vi "run_tests.vi"(11 "Command Line":string[](array[string])) -> (2 "stdout | stderr":string, 3 "Return Code":i32)   [LabVIEW 2021]
uses:
  <vilib>/Utility/error.llb/DialogType.ctl
  20ab466a-1420-47d7-bd04-4ec556d045c0.vi
  <vilib>/Utility/error.llb/Error Cluster From Error Code.vi
  <vilib>/Comparison/Equal/Equal Functor/Equal Functor.lvclass
  <vilib>/ErrorRing/Error Ring.xnode
panel:
  out "Any Failures?":bool
  out "Live results":string
  out "Current Test\nSucceeded":bool
  out "Current":i32
  out "Total":i32
  out "Current Test":path
  out "Full Report":string
  out "All Tests Passed":bool
  out "error out":errorcluster
  # "Required by LabVIEWCLI\n(via connector pane)"
  # "Of"
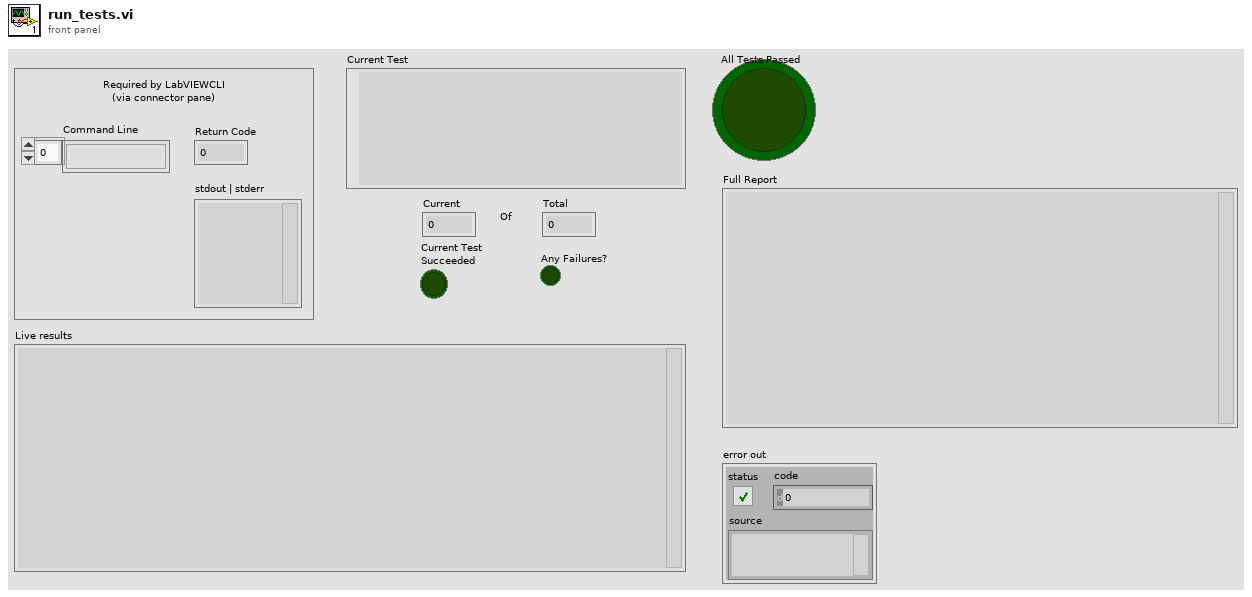
[diagram p1: front panel]
types:
  T1 = typedef "DialogType.ctl" = u16
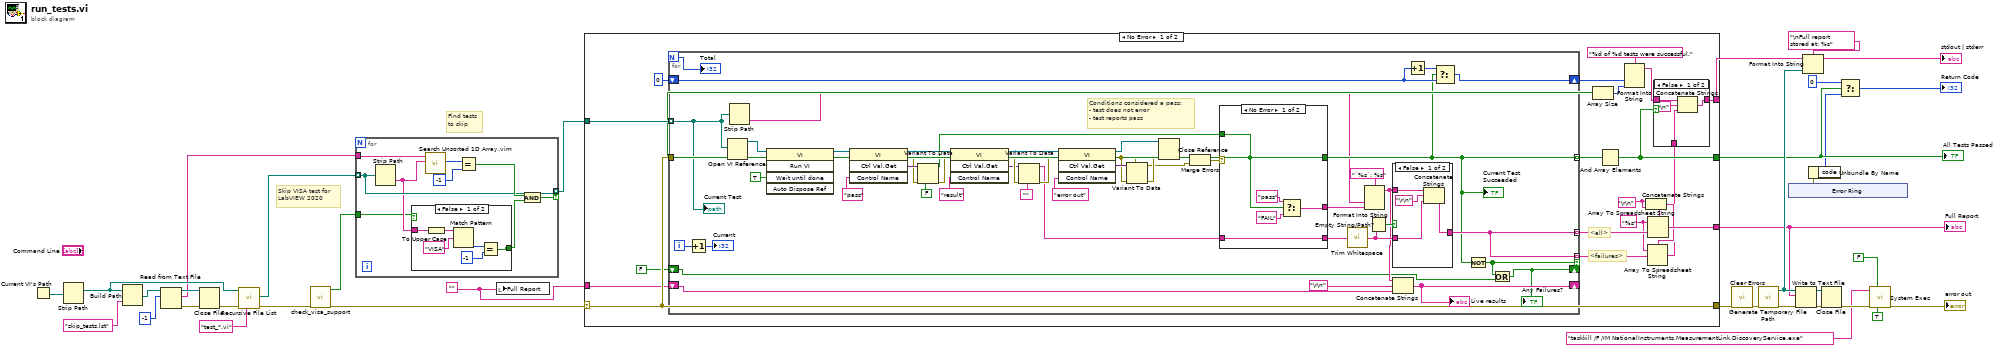
[diagram p0: block diagram]
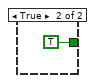
[diagram p2: hidden frame]
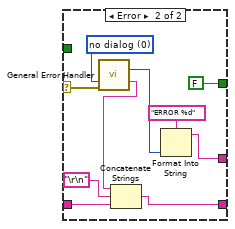
[diagram p5: hidden frame]
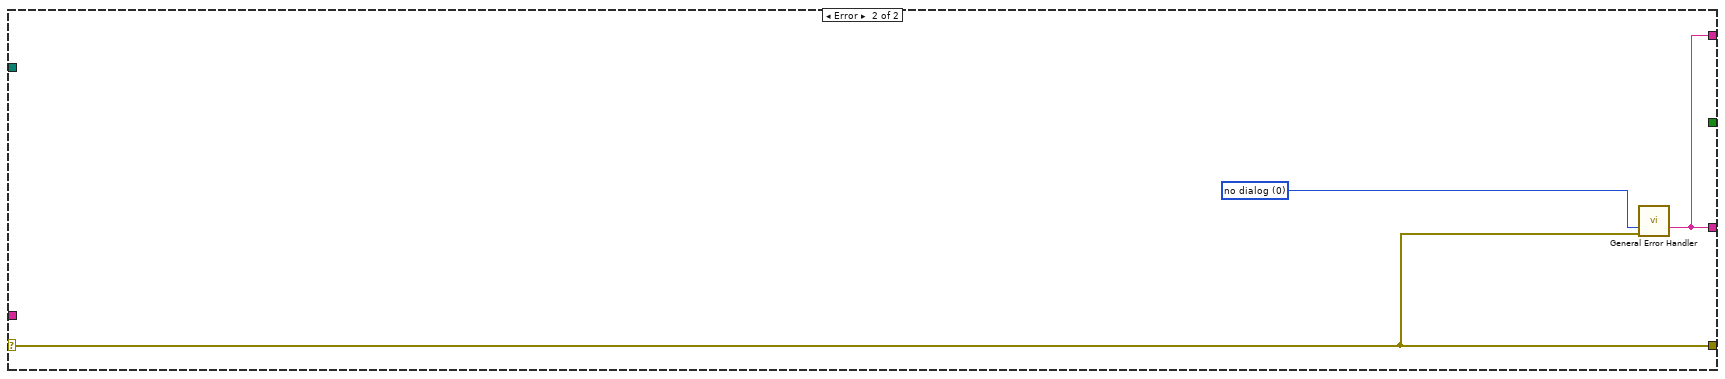
[diagram p6: hidden frame]
diagram:
  w1 = ""
  # "Skip VISA test for LabVIEW 2020"
  # "Find tests\nto skip"
  n1 = Current VI's Path() -> (path=w36:path)
  n2 = Strip Path(path=w36) -> (stripped path=w16:path)  [unwired: 1 out]
  n3 = Build Path(base path=w16, name or relative path="skip_tests.lst") -> (appended path=w14:path)
  n4 = Read from Text File(file (use dialog)=w14, count=-1) -> (refnum out=w17:refnum<file>, text=w11:string[], error out=w19:errorcluster)  [unwired: 2 in, 1 out]
  n5 = Close File(refnum=w17, error in=w19) -> (error out=w18:errorcluster)  [unwired: 1 out]
  n6 = call <vilib>:"Recursive File List.vi"("pattern"="test_*.vi", "error in (no error)"=w18, "Folder Path"=w16) -> ("error out"=w8:errorcluster, "All Files in Dir"=w12:path[])  [unwired: 4 in, 3 out]
  n7 = call "check_visa_support.vi"("error in"=w8) -> ("error out"=w2:errorcluster, "visa supported"=w9:bool)  [unwired: 9 in]
  n8 = for {
    tunnel: w12 -> [w40] mode=indexing
    tunnel: w11 -> [w45]
    tunnel: [w40] -> w10 mode=indexing if=w42
    tunnel: w9 -> [w37]
    n9 = Strip Path(path=w40) -> (name=w38:string)  [unwired: 1 out]
    n10 = case shown="False" w37 {
      tunnel: [w46 TRUE] -> w39
      tunnel: w38 -> [w47 _]
      frame False {
        n11 = To Upper Case(1:w47) -> (0:w51:string)
        n12 = Match Pattern(string=w51, regular expression="VISA") -> (offset past match=w50:i32)  [unwired: 1 in, 3 out]
        n13 = Equal?(x=w50, y=-1) -> (x = y?=w46:bool)
      }
      frame True {
      }
    }
    n14 = call "Search Unsorted 1D Array.vim"("element"=w38, "unsorted 1D array"=w45) -> ("index of element"=w44:i32)  [unwired: 9 in]
    n15 = Equal?(x=w44, y=-1) -> (x = y?=w43:bool)
    n16 = And(x=w43, y=w39) -> (x .and. y?=w42:bool)
  }
  n17 = local write "Full Report"(w1) -> ()
  n18 = case shown="No Error" w2 {
    selector: w2 -> [w70 w149]
    tunnel: w10 -> [w71 _]
    tunnel: [w70 w149] -> w34
    tunnel: [w63 _] -> w25
    tunnel: [w60 w147] -> w26
    tunnel: [w61 w147] -> w31
    tunnel: w1 -> [w54 _]
    frame No Error {
      w56 = "%s" ("format string")
      w69 = "\r\n"
      # "<failures>"
      # "<all>"
      n19 = for {
        N -> [w88]
        tunnel: w71 -> [w89] mode=indexing
        tunnel: w70 -> [w126]
        tunnel: [w91] -> w65 mode=indexing
        tunnel: [w94] -> w59 mode=indexing
        tunnel: [w94] -> w58 mode=indexing if=w79
        shift-right: [w90] -> w66
        shift-left: 0 -> [w92]
        shift-right: [w82] -> _
        shift-left: w54 -> [w81]
        shift-right: [w77] -> _
        shift-left: FALSE -> [w78]
        i -> [w87]
        # "Conditions considered a pass:\n- test does not error\n- test reports pass"
        n20 = Increment(x=w87) -> (x+1=→"Current":i32)
        n21 = Open VI Reference(vi path=w89, error in (no error)=w126) -> (vi reference=w125:refnum<vi>, error out=w124:errorcluster)  [unwired: 4 in]
        n22 = Strip Path(path=w89) -> (name=w85:string)  [unwired: 1 out]
        n23 = invoke class="VI" method="Run VI"(reference=w125, error in=w124, "Wait until done"=TRUE ("Wait Until Done")) -> (reference out=w122:refnum<vi>, error out=w121:errorcluster)  [unwired: 2 in, 3 out]
        n24 = invoke class="VI" method="Ctrl Val.Get"(reference=w122, error in=w121, "Control Name"="pass") -> (reference out=w111:refnum<vi>, error out=w118:errorcluster, "Get Control Value Variant"=w119:variant)  [unwired: 1 in, 1 out]
        n25 = Variant To Data(error in=w118, type=FALSE, Variant=w119) -> (data=w100:bool, error out=w115:errorcluster)
        n26 = invoke class="VI" method="Ctrl Val.Get"(reference=w111, error in=w115, "Control Name"="result") -> (reference out=w106:refnum<vi>, error out=w116:errorcluster, "Get Control Value Variant"=w113:variant)  [unwired: 1 in, 1 out]
        n27 = Variant To Data(error in=w116, type="", Variant=w113) -> (data=w98:string, error out=w109:errorcluster)
        n28 = invoke class="VI" method="Ctrl Val.Get"(reference=w106, error in=w109, "Control Name"="error out") -> (reference out=w105:refnum<vi>, error out=w107:errorcluster, "Get Control Value Variant"=w110:variant)  [unwired: 1 in, 1 out]
        n29 = Variant To Data(error in=w107, type=w107, Variant=w110) -> (data=w102:errorcluster, error out=w108:errorcluster)
        n30 = Close Reference(reference=w105, error in (no error)=w108) -> (error out=w103:errorcluster)
        n31 = Merge Errors(w103, w102) -> (w101:errorcluster)
        n32 = case shown="No Error" w101 {
          selector: w101 -> [_ w144]
          tunnel: w100 -> [w134 _]
          tunnel: [w133 w141] -> w84
          tunnel: [w134 FALSE] -> w91
          tunnel: w98 -> [w132 w140]
          tunnel: [w132 w139] -> w97
          frame No Error {
            n33 = Select(t="pass" ("Control Name"), s=w134, f="FAIL" ("Control Name")) -> (s? t:f=w133:string)
          }
          frame Error {
            w145 = T1 0 items=["no dialog", "OK message", "continue or stop message", "OK message + warnings", "continue/stop + warnings"] ("type of dialog (OK msg:1)")
            n34 = call <vilib>:"General Error Handler.vi"("type of dialog (OK msg:1)"=w145, "error in (no error)"=w144) -> ("code out"=w143:i32, "message"=w138:string)  [unwired: 9 in, 3 out]
            n35 = Concatenate Strings(w138, "\r\n", w140) -> (w139:string)
            n36 = Format Into String(format string="ERROR %d", w143) -> (resulting string=w141:string)  [unwired: 2 in, 1 out]
          }
        }
        "Current Test\nSucceeded" <- w91
        n37 = call <vilib>:"Trim Whitespace.vi"("string"=w97) -> ("trimmed string"=w96:string)  [unwired: 1 in]
        n38 = Format Into String(format string="`%s`: %s" ("Control Name"), w85, w84) -> (resulting string=w80:string)  [unwired: 2 in, 1 out]
        n39 = Empty String/Path?(string/path=w96) -> (empty?=w95:bool)
        n40 = case shown="False" w95 {
          tunnel: w96 -> [w129 _]
          tunnel: w80 -> [w130 w131]
          tunnel: [w128 w131] -> w94
          frame False {
            n41 = Concatenate Strings(w130, "\r\n", w129) -> (w128:string)
          }
          frame True {
          }
        }
        n42 = Concatenate Strings(w80, "\r\n", w81) -> (w82:string)
        "Live results" <- w82
        n43 = Increment(x=w92) -> (x+1=w93:i32)
        n44 = Select(t=w93, s=w91, f=w92) -> (s? t:f=w90:i32)
        n45 = Not(x=w91) -> (.not. x?=w79:bool)
        n46 = Or(x=w79, y=w78) -> (x .or. y?=w77:bool)
        "Any Failures?" <- w77
        "Current Test" <- w89
        "Total" <- w88
      }
      n47 = Array Size(array=w65) -> (size(s)=w64:i32)
      n48 = And Array Elements(Boolean array=w65) -> (logical AND=w63:bool)
      n49 = Format Into String(format string="%d of %d tests were successful." ("Control Name"), w66, w64) -> (resulting string=w62:string)  [unwired: 2 in, 1 out]
      n50 = Concatenate Strings(w69, w69) -> (w57:string)
      n51 = Array To Spreadsheet String(delimiter (Tab)=w57, array=w58, 3:w56) -> (spreadsheet string=w55:string)
      n52 = Array To Spreadsheet String(delimiter (Tab)=w57, array=w59, 3:w56) -> (spreadsheet string=w60:string)
      n53 = case shown="False" w63 {
        tunnel: w62 -> [w75 w76]
        tunnel: [w72 w76] -> w61
        tunnel: w55 -> [w73 _]
        frame False {
          n54 = Concatenate Strings(w75, "\r\n", w73) -> (w72:string)
        }
        frame True {
        }
      }
    }
    frame Error {
      w148 = T1 0 items=["no dialog", "OK message", "continue or stop message", "OK message + warnings", "continue/stop + warnings"] ("type of dialog (OK msg:1)")
      n55 = call <vilib>:"General Error Handler.vi"("type of dialog (OK msg:1)"=w148, "error in (no error)"=w149) -> ("message"=w147:string)  [unwired: 9 in, 4 out]
    }
  }
  "All Tests Passed" <- w25
  "Full Report" <- w26
  n56 = call <vilib>:"Clear Errors.vi"("error in (no error)"=w34) -> ("error out"=w33:errorcluster)  [unwired: 5 in, 1 out]
  n57 = call <vilib>:"Generate Temporary File Path.vi"("error in (no error)"=w33) -> ("error out"=w28:errorcluster, "Unique Temporary File Path"=w29:path)  [unwired: 9 in]
  n58 = xnode "Error Ring"() -> ("error out"=w21:errorcluster)
  n59 = Write to Text File(file (use dialog)=w29, text=w26, error in=w28) -> (refnum out=w30:refnum<file>, error out=w27:errorcluster)  [unwired: 1 in, 1 out]
  n60 = Format Into String(format string="\nFull report stored at: %s" ("Control Name"), initial string=w31, w29) -> (resulting string=→"stdout | stderr":string)  [unwired: 1 in, 1 out]
  n61 = Unbundle By Name(w21) -> ("code"=w20:i32)
  n62 = Close File(refnum=w30, error in=w27) -> (error out=w7:errorcluster)  [unwired: 1 out]
  n63 = Select(t=0, s=w25, f=w20) -> (s? t:f=→"Return Code":i32)
  n64 = call <vilib>:"System Exec.vi"("run minimized? (F)"=TRUE, "wait until completion? (T)"=FALSE, "error in (no error)"=w7, "command line"="taskkill /F /IM NationalInstruments.MeasurementLink.DiscoveryService.exe") -> ("error out"=→"error out":errorcluster)  [unwired: 4 in, 3 out]
